vi "DAC Init Results.vi"(8 "error in":errorcluster, 9 "Log Details?":bool, 10 "tdms file":refnum<k34>, 11 "DAC Inclino in":refnum<class "DAC Inclinometer.lvclass">) -> (0 "error out":errorcluster, 2 "tdms file out":refnum<k34>)   [LabVIEW 2019, in "DAC.lvlib" / "DAC Inclinometer.lvclass"]
uses:
  DAC Inclinometer.lvclass
  C:/Users/wg/Documents/LV_Projects/test-stand/App/DAC/DAC.lvclass
  DAC.lvclass/DAC.ctl
  DAC Inclinometer.lvclass/DAC Inclinometer.ctl
  DAC.lvclass
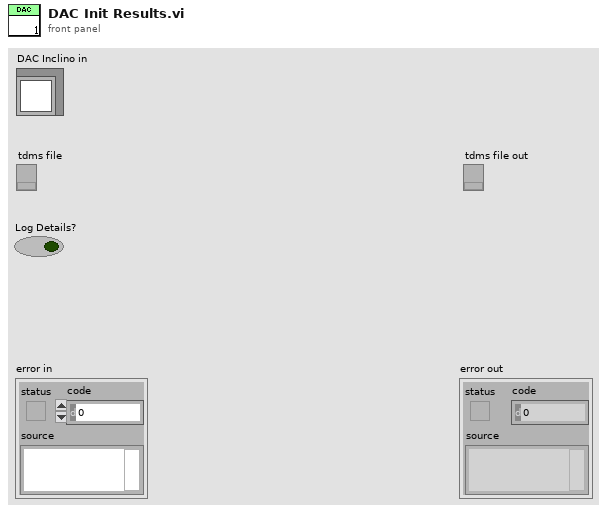
[diagram p1: front panel]
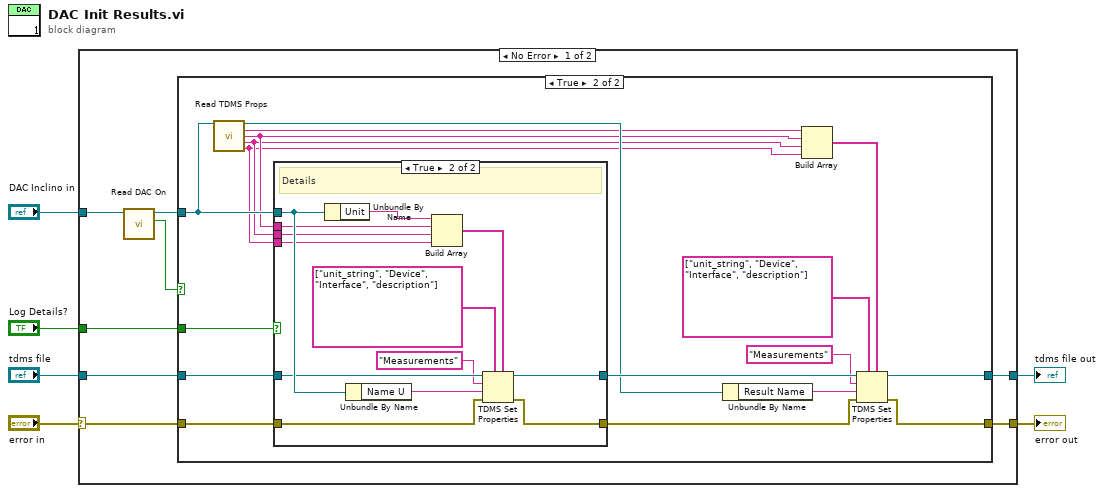
[diagram p0: block diagram]
diagram:
  n1 = case shown="No Error" "error in" {
    selector: "error in" -> [w7 w50]
    tunnel: [w9 w50] -> w6
    tunnel: "DAC Inclino in" -> [w8 _]
    tunnel: "tdms file" -> [w12 w49]
    tunnel: [w10 w49] -> w5
    tunnel: "Log Details?" -> [w11 _]
    frame No Error {
      n2 = call "Read DAC On.vi"("DAC in"=w8) -> ("DAC On"=w13:bool, "DAC out"=w14:refnum<class "DAC Inclinometer.lvclass">)  [unwired: 8 in, 1 out]
      n3 = case shown="True" w13 {
        tunnel: w12 -> [w16 w31]
        tunnel: [w16 w28] -> w10
        tunnel: [w15 w27] -> w9
        tunnel: w14 -> [_ w22]
        tunnel: w11 -> [_ w32]
        tunnel: w7 -> [w15 w23]
        frame False {
        }
        frame True {
          n4 = call "Read TDMS Props.vi"("DAC in"=w22) -> ("DAC out"=w21:refnum<class "DAC Inclinometer.lvclass">, "Result Unit"=w20:string, "DAC Device"=w19:string, "DAC IO"=w18:string, "DAC Description"=w17:string)  [unwired: 10 in]
          n5 = case shown="True" w32 {
            tunnel: w31 -> [w35 w45]
            tunnel: [w35 w44] -> w29
            tunnel: [w34 w40] -> w30
            tunnel: w22 -> [_ w47]
            tunnel: w23 -> [w34 w36]
            tunnel: w19 -> [_ w39]
            tunnel: w18 -> [_ w38]
            tunnel: w17 -> [_ w37]
            frame False {
            }
            frame True {
              # "Details"
              n6 = Unbundle By Name(w47) -> ("Unit"=w48:string)
              n7 = Unbundle By Name(w47) -> ("Name U"=w46:string)
              n8 = Build Array(w48, w39, w38, w37) -> (w41:string[])
              n9 = TDMS Set Properties(5:w41, 7:string[] ["unit_string", "Device", "Interface", "description"] ("property names"), 8:w36, 9:w46, 10:"Measurements" ("group name in (Untitled)"), 11:w45) -> (0:w40:errorcluster, 3:w44:refnum<k34>)  [unwired: 2 out]
            }
          }
          n10 = Unbundle By Name(w21) -> ("Result Name"=w33:string)
          n11 = Build Array(w20, w19, w18, w17) -> (w24:string[])
          n12 = TDMS Set Properties(5:w24, 7:string[] ["unit_string", "Device", "Interface", "description"] ("property names"), 8:w30, 9:w33, 10:"Measurements" ("group name in (Untitled)"), 11:w29) -> (0:w27:errorcluster, 3:w28:refnum<k34>)  [unwired: 2 out]
        }
      }
    }
    frame Error {
    }
  }
  "error out" <- w6
  "tdms file out" <- w5
